vi "MaybeFinally TF.vi"() -> ()   [LabVIEW 2025]
uses:
  <vilib>/express/express arith-compare/Formula/XNode/ExpressFormulaBlockNode.xnode
panel:
  out "LOG":string
  out "TEMP":dbl(slide) scale=0.0..60.0
  out "PWM":dbl(knob) scale=0.0..255.0
  out "read buffer":string
  in  "VISA resource name":refnum<visa-resource-name>
  in  "byte count":u32
  in  "stop":bool
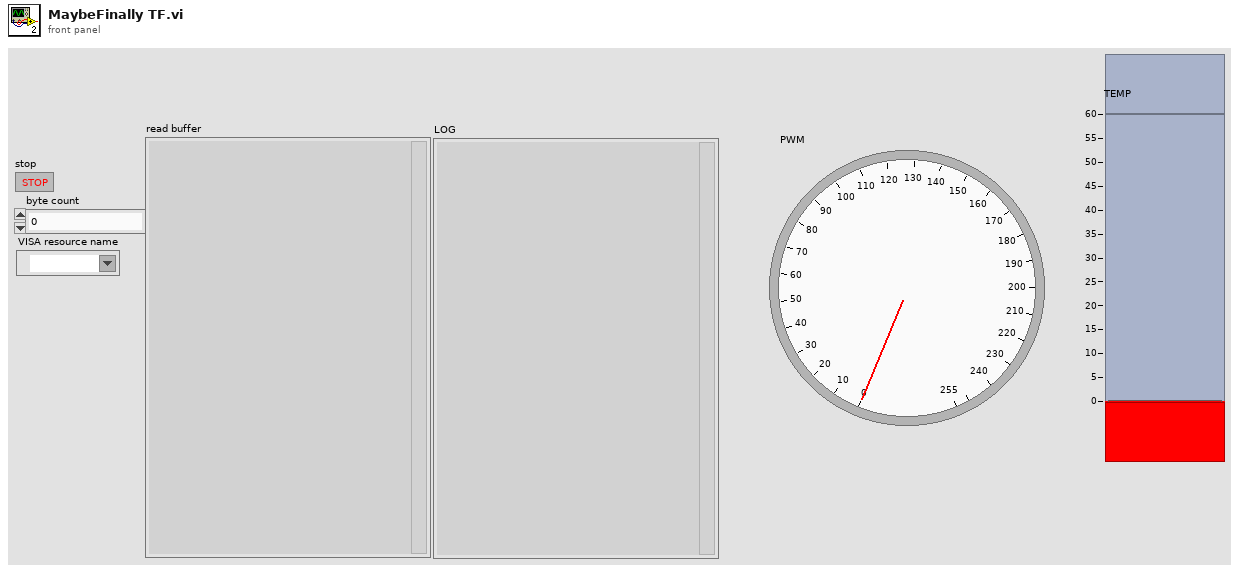
[diagram p1: front panel]
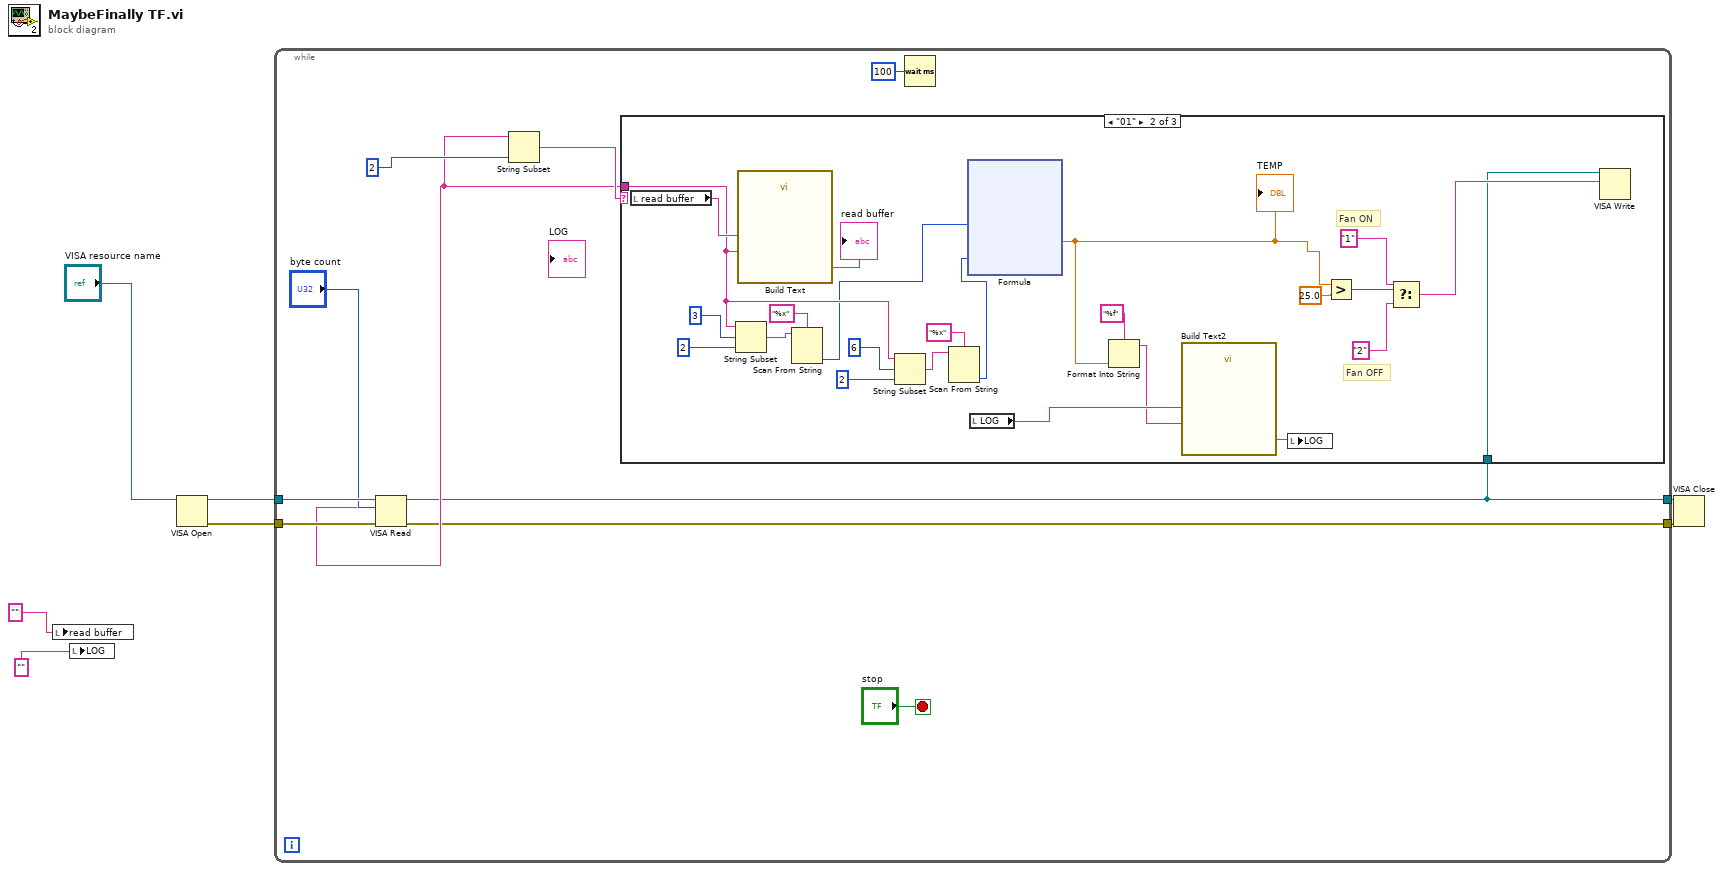
[diagram p0: block diagram]
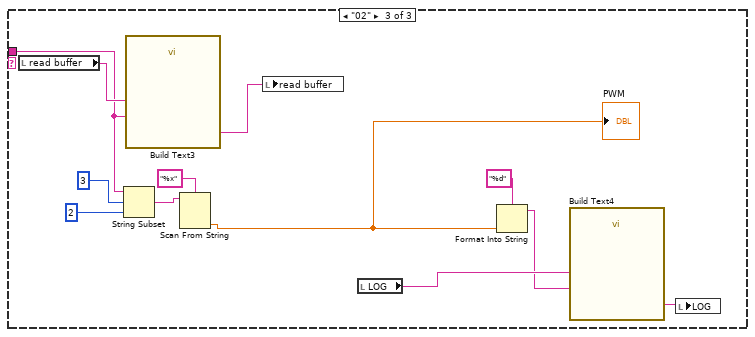
[diagram p3: hidden frame]
diagram:
  n1 = local write "read buffer"("" ("read buffer")) -> ()
  n2 = local write "LOG"("" ("LOG")) -> ()
  n3 = VISA Open(VISA resource name="VISA resource name") -> (VISA resource name=w7:refnum<visa-resource-name>, error out=w6:errorcluster)  [unwired: 4 in]
  n4 = while {
    tunnel: w7 -> [w15]
    tunnel: w6 -> [w14]
    tunnel: [w8] -> w5
    tunnel: [w9] -> w4
    stop <- "stop" stop-if-true
    n5 = VISA Read(VISA resource name=w15, byte count="byte count", error in (no error)=w14) -> (VISA resource name out=w8:refnum<visa-resource-name>, read buffer=w10:string, error out=w9:errorcluster)  [unwired: 1 out]
    n6 = String Subset(string=w10, length (rest)=2 ("length (rest)")) -> (substring=w11:string)  [unwired: 1 in]
    n7 = case shown="\"01\"" w11 {
      tunnel: w10 -> [_ w35 w54]
      tunnel: w8 -> [_ w18 _]
      frame "False", Default {
      }
      frame "01" {
        # "Fan ON"
        # "Fan OFF"
        n8 = local read "read buffer"() -> (w41:string)
        n9 = String Subset(string=w35, offset (0)=3, length (rest)=2 ("length (rest)")) -> (substring=w34:string)
        n10 = call "Build Text"("old"=w41, "new"=w35) -> ("Result"=→"read buffer":string)  [unwired: 12 in, 1 out]
        n11 = Scan From String(format string="%x", input string=w34) -> (output 1=w32:u32)  [unwired: 3 in, 3 out]
        n12 = String Subset(string=w35, offset (0)=6, length (rest)=2 ("length (rest)")) -> (substring=w31:string)
        n13 = Scan From String(format string="%x", input string=w31) -> (output 1=w29:u32)  [unwired: 3 in, 3 out]
        n14 = xnode "Formula"("X1"=w32, "X2"=w29) -> ("Result"=w20:dbl)  [unwired: 1 in, 1 out]
        "TEMP" <- w20
        n15 = local read "LOG"() -> (w28:string)
        n16 = Format Into String(format string="%f", w20) -> (resulting string=w26:string)  [unwired: 2 in, 1 out]
        n17 = call "Build Text2"("old"=w28, "temp"=w26) -> ("Result"=w25:string)  [unwired: 12 in, 1 out]
        n18 = local write "LOG"(w25) -> ()
        n19 = Greater?(x=w20, y=25.0) -> (0:w24:bool)
        n20 = Select(t="1", s=w24, f="2") -> (s? t:f=w21:string)
        n21 = VISA Write(VISA resource name=w18, write buffer=w21) -> ()  [unwired: 1 in, 3 out]
      }
      frame "02" {
        n22 = local read "read buffer"() -> (w63:string)
        n23 = String Subset(string=w54, offset (0)=3, length (rest)=2 ("length (rest)")) -> (substring=w60:string)
        n24 = call "Build Text3"("old"=w63, "new"=w54) -> ("Result"=w52:string)  [unwired: 12 in, 1 out]
        n25 = Scan From String(format string="%x", input string=w60) -> (output 1=w53:dbl)  [unwired: 3 in, 3 out]
        "PWM" <- w53
        n26 = local write "read buffer"(w52) -> ()
        n27 = local read "LOG"() -> (w58:string)
        n28 = Format Into String(format string="%d", w53) -> (resulting string=w56:string)  [unwired: 2 in, 1 out]
        n29 = call "Build Text4"("old"=w58, "pwm"=w56) -> ("Result"=w55:string)  [unwired: 12 in, 1 out]
        n30 = local write "LOG"(w55) -> ()
      }
    }
    n31 = Wait (ms)(milliseconds to wait=u32 100) -> ()  [unwired: 1 out]
  }
  n32 = VISA Close(VISA resource name=w5, error in (no error)=w4) -> ()  [unwired: 1 out]
